vi "Test Streaming.vi"() -> ()   [LabVIEW 2021]
uses:
  CAN RW CANsub.lvclass
  <vilib>/CIF Foundation/CIF CAN RW Core/CAN_RW_CORE.lvclass
  <vilib>/CIF Foundation/CIF PCAP Parse and Build/pcap_Parse_Build_CIF.lvclass
  <vilib>/CIF Foundation/CIF PCAP Parse and Build/Typedef/Format Specific/CAN Interface Mode.ctl
  <vilib>/CIF Foundation/CIF PCAP Parse and Build/Typedef/Format Specific/CAN Metadata.ctl
  <vilib>/CIF Foundation/CIF CAN RW Core/typedef/CAN Mode.ctl
  <vilib>/CIF Foundation/CIF CAN RW Core/typedef/FD Config.ctl
  <vilib>/CIF Foundation/CIF CAN RW Core/typedef/CAN Port Configuration.ctl
  <vilib>/CIF Foundation/CIF CAN RW Core/typedef/CAN Filter.ctl
  <vilib>/CIF Foundation/CIF CAN RW Core/typedef/Statistics.ctl
panel:
  out "writer stats":T1
  out "reader stats":T1
  out "rx payloads":u8[][](array[numeric]) format="%.0x"
  out "rx metadata":T2[](array[typedef]) {"identifier" format="%.0x"}
  out "error out":errorcluster
  out "Timeout":bool[](array[boolean])
  out "number read":i32[](array[numeric])
  out "number written":i32
  in  "cut last packet":bool
  in  "number to read":i32=100
  in  "reader filter":T4 {"Deny List (ID)" format="%.0x"; "Allow List (ID)" format="%.0x"}
  in  "Port Configuration":T5={"Mode"=enum."CAN FD", "Baud Rate"=500000, "Temination On"=TRUE, "Subordinate"=FALSE, "Echo TX"=FALSE, "FD Config"={"FD Baud Rate"=2000000, "ISO Mode"=TRUE, "BRS Enabled"=TRUE}} {"FD Config"."FD Baud Rate" format="%.0p"; "Baud Rate" format="%.0p"}
  in  "reader interface":string="192.168.0.49/2"
  in  "write interface":string="192.168.0.49/1"
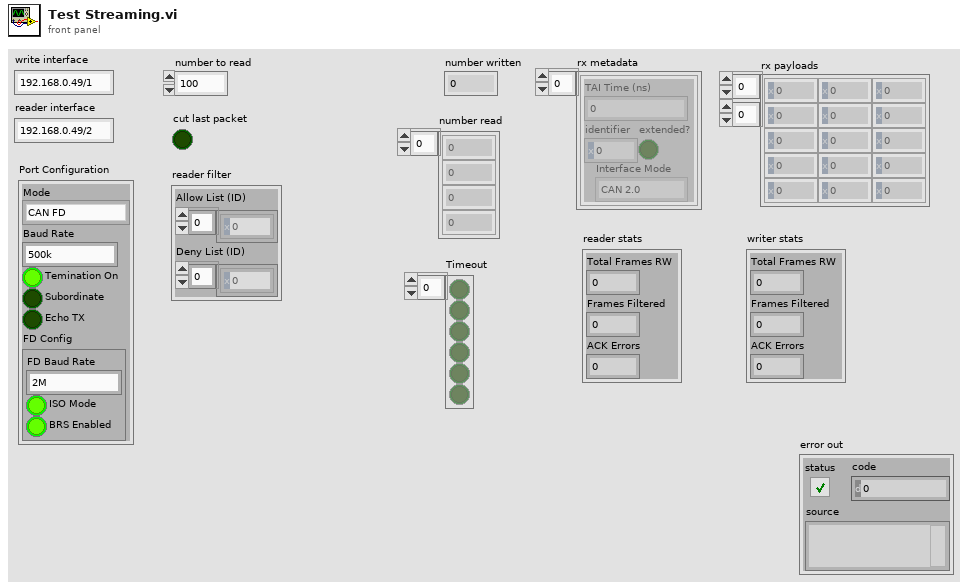
[diagram p1: front panel]
types:
  T1 = typedef "CAN_RW_CORE.lvclass/Statistics.ctl" = cluster{"Total Frames RW":u32, "Frames Filtered ":u32, "ACK Errors":u32}
  T2 = typedef "pcap_Parse_Build_CIF.lvclass/CAN Metadata.ctl" = cluster{"TAI Time (ns)":i64, "identifier":u32, "extended?":bool, "Interface Mode":T3}
  T3 = typedef "pcap_Parse_Build_CIF.lvclass/CAN Interface Mode.ctl" = enum16{"CAN 2.0", "CAN FD", "CAN FD BRS", "Remote"}
  T4 = typedef "CAN_RW_CORE.lvclass/CAN Filter.ctl" = cluster{"Allow List (ID)":u32[], "Deny List (ID)":u32[]}
  T5 = typedef "CAN_RW_CORE.lvclass/CAN Port Configuration.ctl" = cluster{"Mode":T6, "Baud Rate":u64, "Temination On":bool, "Subordinate":bool, "Echo TX":bool, "FD Config":T7}
  T6 = typedef "CAN_RW_CORE.lvclass/CAN Mode.ctl" = enum16{"CAN 2.0", "CAN FD"}
  T7 = typedef "CAN_RW_CORE.lvclass/FD Config.ctl" = cluster{"FD Baud Rate":u64, "ISO Mode":bool, "BRS Enabled":bool}
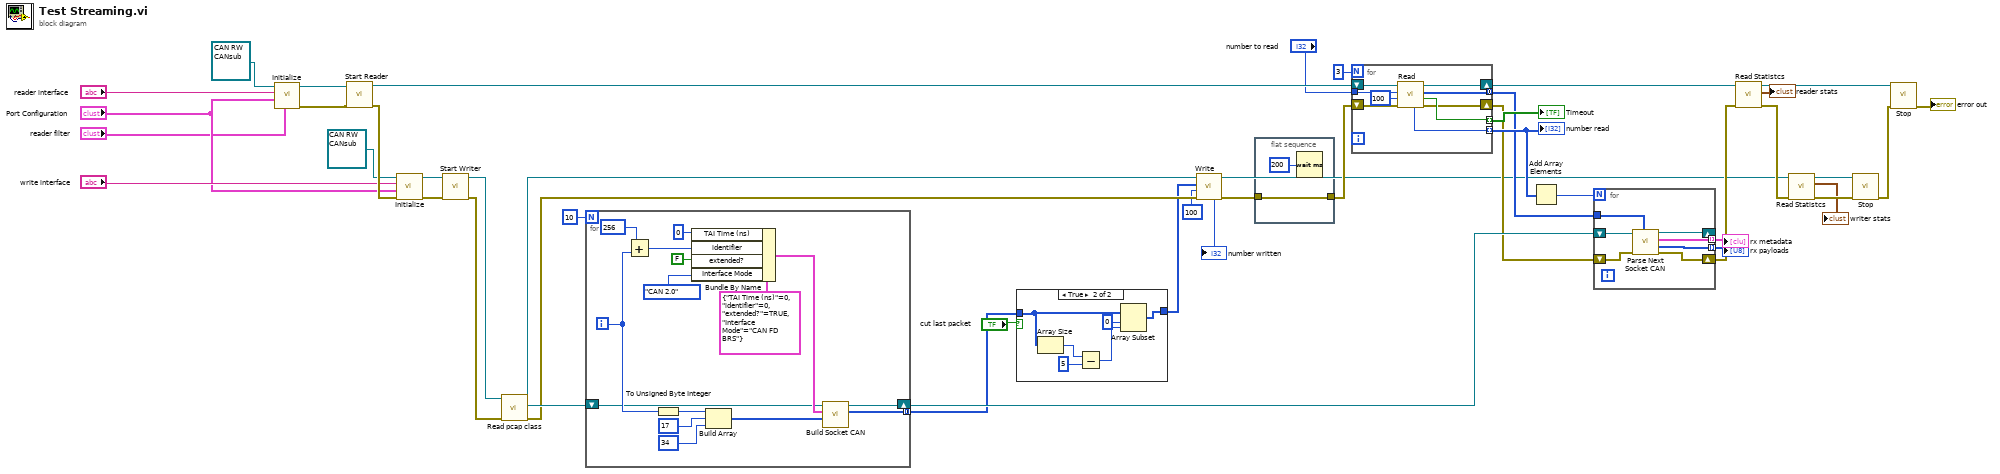
[diagram p0: block diagram]
diagram:
  n1 = call "Initialize.vi"("Filter"="reader filter", "Port Configuration"="Port Configuration", "Interface"="reader interface", "CANsub_CAN_RW in"=refnum<class "CAN RW CANsub.lvclass"> refnum ("CAN RW CANsub.lvclass")) -> ("error out"=w46:errorcluster, "CANsub_CAN_RW out"=w42:refnum<class "CAN RW CANsub.lvclass">)  [unwired: 6 in]
  n2 = call-dynamic "Start Reader.vi"("error in (no error)"=w46, "CAN RW CANsub in"=w42) -> ("error out"=w45:errorcluster, "CAN RW CANsub out"=w25:refnum<class "CAN RW CANsub.lvclass">)  [unwired: 8 in]
  n3 = call "Initialize.vi"("error in (no error)"=w45, "Port Configuration"="Port Configuration", "Interface"="write interface", "CANsub_CAN_RW in"=refnum<class "CAN RW CANsub.lvclass"> refnum ("CAN RW CANsub.lvclass")) -> ("error out"=w44:errorcluster, "CANsub_CAN_RW out"=w35:refnum<class "CAN RW CANsub.lvclass">)  [unwired: 6 in]
  n4 = call-dynamic "Start Writer.vi"("error in (no error)"=w44, "CAN RW CANsub in"=w35) -> ("error out"=w33:errorcluster, "CAN RW CANsub out"=w36:refnum<class "CAN RW CANsub.lvclass">)  [unwired: 8 in]
  n5 = call <vilib>:"Read pcap class.vi"("error in (no error)"=w33, "CAN_RW_CORE in"=w36) -> ("error out"=w31:errorcluster, "pcap class"=w32:refnum<class "pcap_Parse_Build_CIF.lvclass">, "CAN_RW_CORE out"=w30:refnum<class "CAN RW CANsub.lvclass">)  [unwired: 7 in]
  n6 = for {
    N: 10 -> [_]
    shift-right: [w48] -> w19
    shift-left: w32 -> [w50]
    tunnel: [w47] -> w2 mode=concatenating
    i -> [w54]
    n7 = Add(x=u32 256, y=w54) -> (x+y=w58:u32)
    n8 = To Unsigned Byte Integer(number=w54) -> (unsigned 8bit integer=w53:u8)
    n9 = Bundle By Name(cluster=T2 {"TAI Time (ns)"=0, "identifier"=0, "extended?"=TRUE, "Interface Mode"=enum."CAN FD BRS"} ("CAN Metadata"), "TAI Time (ns)"=i64 0, "identifier"=w58, "extended?"=FALSE, "Interface Mode"=CAN_Interface_Mode."CAN 2.0") -> (w55:T2)
    n10 = Build Array(w53, u8 17, u8 34) -> (w49:u8[])
    n11 = call <vilib>:"Build Socket CAN.vi"("Payload"=w49, "CAN Metadata"=w55, "pcap Parse and Build in"=w50) -> ("CAN Packet"=w47:u8[], "pcap Parse and Build out"=w48:refnum<class "pcap_Parse_Build_CIF.lvclass">)  [unwired: 7 in]
  }
  n12 = case shown="True" "cut last packet" {
    tunnel: [w62 w64] -> w1
    tunnel: w2 -> [w62 w66]
    frame False {
    }
    frame True {
      n13 = Array Size(array=w66) -> (size(s)=w68:i32)
      n14 = Subtract(x=w68, y=5) -> (x-y=w65:i32)
      n15 = Array Subset(array=w66, index=0, length=w65) -> (w64:u8[])
    }
  }
  n16 = call-dynamic "Write.vi"("error in (no error)"=w31, "timeout (ms)"=100, "pcap CAN DATA in"=w1, "CAN RW CANsub in"=w30) -> ("error out"=w27:errorcluster, "CAN RW CANsub out"=w6:refnum<class "CAN RW CANsub.lvclass">, "number written"=→"number written":i32)  [unwired: 5 in]
  n17 = flat-sequence {
    tunnel: w27 -> [w69]
    tunnel: [w69] -> w24
    frame #0 {
      n18 = Wait (ms)(milliseconds to wait=u32 200) -> ()  [unwired: 1 out]
    }
  }
  n19 = for {
    N: 3 -> [_]
    shift-right: [w72] -> w16
    shift-left: w25 -> [w79]
    shift-right: [w71] -> w17
    shift-left: w24 -> [w78]
    tunnel: "number to read" -> [w77]
    tunnel: [w75] -> w18 mode=concatenating
    tunnel: [w74] -> w21 mode=indexing
    tunnel: [w73] -> w22 mode=indexing
    n20 = call-dynamic "Read.vi"("error in (no error)"=w78, "timeout (ms)"=100, "number to read"=w77, "CAN RW CANsub in"=w79) -> ("error out"=w71:errorcluster, "Timeout"=w73:bool, "pcap CAN Data"=w75:u8[], "CAN RW CANsub out"=w72:refnum<class "CAN RW CANsub.lvclass">, "number read"=w74:i32)  [unwired: 3 in]
  }
  "number read" <- w21
  "Timeout" <- w22
  n21 = Add Array Elements(numeric array=w21) -> (sum=w20:i32)
  n22 = for {
    N: w20 -> [_]
    shift-right: [w85] -> _
    shift-left: w19 -> [w86]
    tunnel: w18 -> [w84]
    tunnel: [w83] -> w11 mode=indexing
    tunnel: [w82] -> w10 mode=indexing
    shift-right: [w80] -> w12
    shift-left: w17 -> [w81]
    n23 = call <vilib>:"Parse Next Socket CAN.vi"("CAN pcap in"=w84, "error in (no error)"=w81, "pcap Parse and Build in"=w86) -> ("error out"=w80:errorcluster, "Payload"=w82:u8[], "CAN Metadata"=w83:T2, "pcap Parse and Build out"=w85:refnum<class "pcap_Parse_Build_CIF.lvclass">)  [unwired: 4 in, 1 out]
  }
  "rx metadata" <- w11
  "rx payloads" <- w10
  n24 = call <vilib>:"Read Statistcs.vi"("error in (no error)"=w12, "CAN_RW_CORE in"=w16) -> ("error out"=w7:errorcluster, "Statistcs"=→"reader stats":T1, "CAN_RW_CORE out"=w14:refnum<class "CAN RW CANsub.lvclass">)  [unwired: 7 in]
  n25 = call <vilib>:"Read Statistcs.vi"("error in (no error)"=w7, "CAN_RW_CORE in"=w6) -> ("error out"=w9:errorcluster, "Statistcs"=→"writer stats":T1, "CAN_RW_CORE out"=w8:refnum<class "CAN RW CANsub.lvclass">)  [unwired: 7 in]
  n26 = call-dynamic "Stop.vi"("error in (no error)"=w9, "CAN RW CANsub in"=w8) -> ("error out"=w15:errorcluster)  [unwired: 8 in, 1 out]
  n27 = call-dynamic "Stop.vi"("error in (no error)"=w15, "CAN RW CANsub in"=w14) -> ("error out"=→"error out":errorcluster)  [unwired: 8 in, 1 out]
